vi "Mode Registration.vi"(8 "error in":errorcluster, 9 "mode":T1=-1 items=["Digital Input"=0, "Digital Output"=1, "Analog Input"=2, "PWM Input"=3, "PWM Output"=4, "Counter Rising"=5, "Counter Falling"=6, "Quadrature"=7, "Addressable LEDs"=13], 10 "device ID":i32=-1, 11 "Action":enum16{"Get", "Set", "Force", "Clear"}(ring)) -> (0 "error out":errorcluster, 2 "mode out":T1 items=["Digital Input"=0, "Digital Output"=1, "Analog Input"=2, "PWM Input"=3, "PWM Output"=4, "Counter Rising"=5, "Counter Falling"=6, "Quadrature"=7, "Addressable LEDs"=13])   [LabVIEW 2023]
uses:
  <vilib>/MRC/Types/MRC Smart IO Mode.ctl
  <vilib>/MRC/MrcLib.lvlib
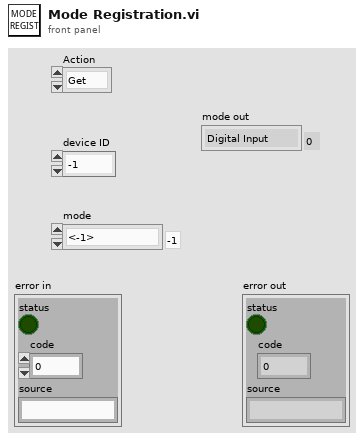
[diagram p1: front panel]
types:
  T1 = typedef "MRC Smart IO Mode.ctl" = i32
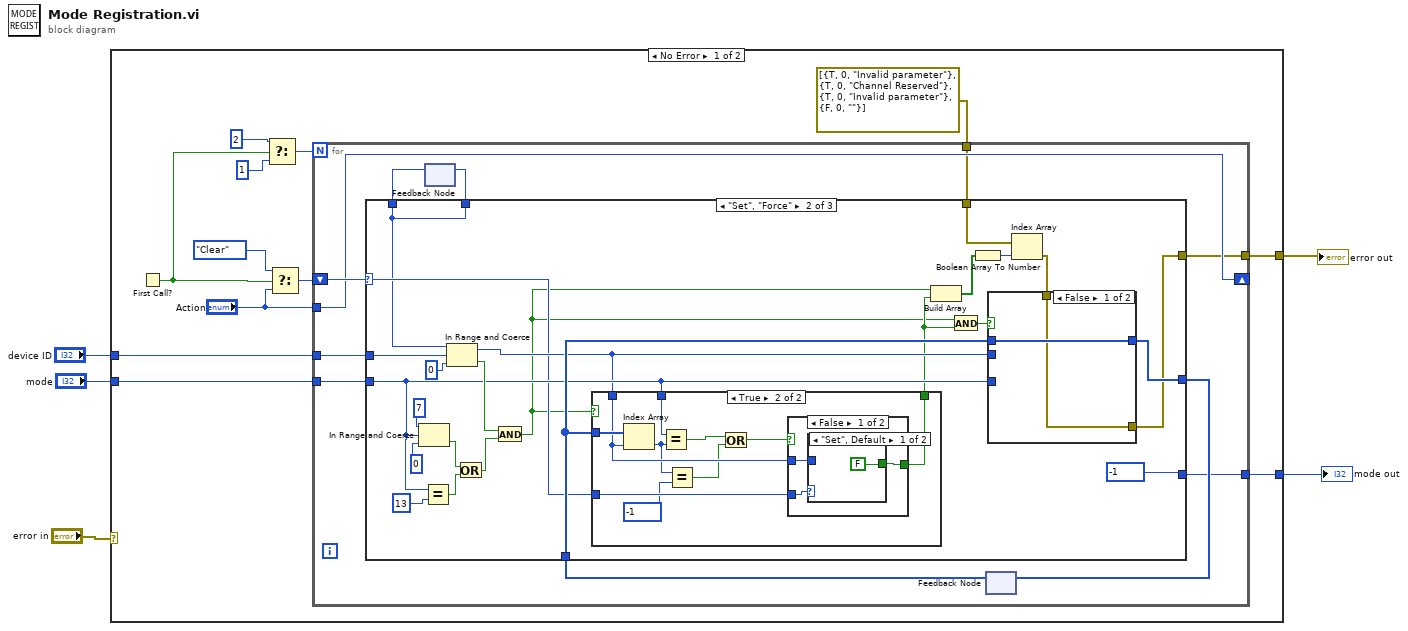
[diagram p0: block diagram]
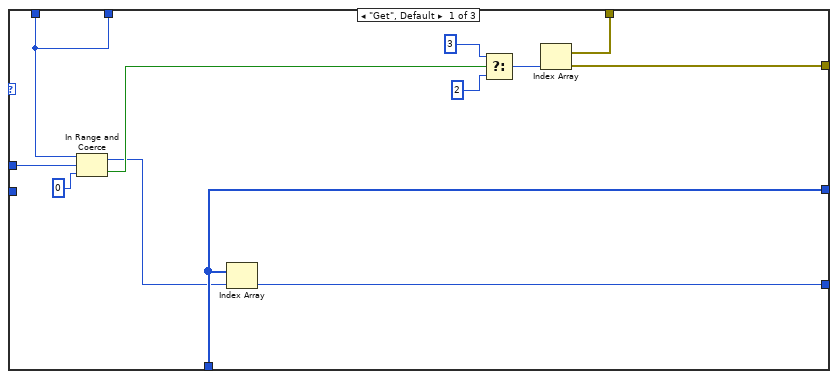
[diagram p2: hidden frame]
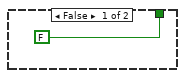
[diagram p3: hidden frame]
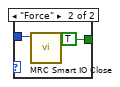
[diagram p4: hidden frame]
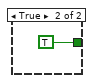
[diagram p5: hidden frame]
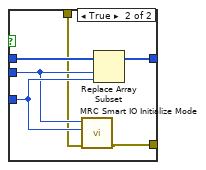
[diagram p6: hidden frame]
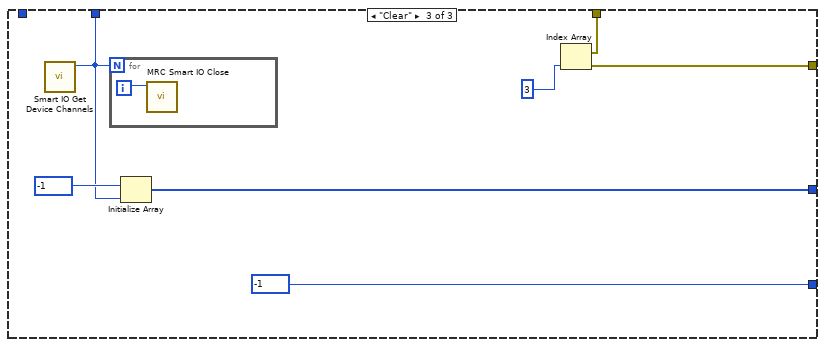
[diagram p7: hidden frame]
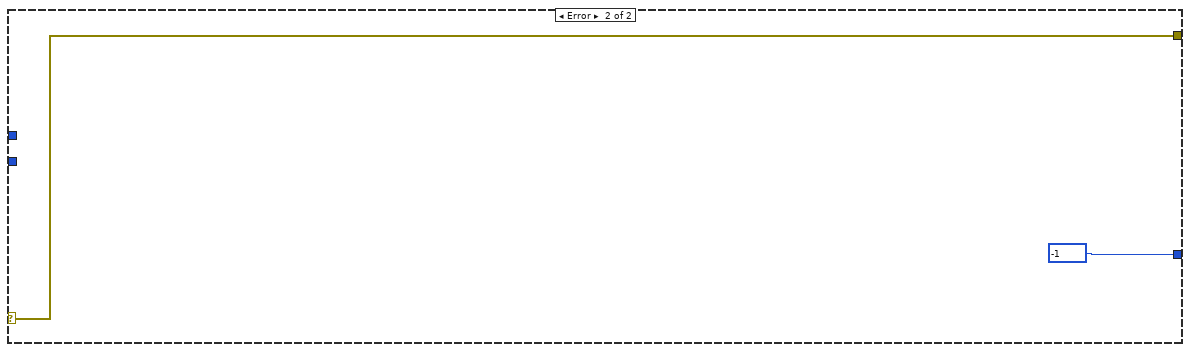
[diagram p8: hidden frame]
diagram:
  n1 = case shown="No Error" "error in" {
    selector: "error in" -> [_ w100]
    tunnel: "device ID" -> [w17 _]
    tunnel: "mode" -> [w16 _]
    tunnel: [w13 w99] -> w3
    tunnel: [w7 w100] -> w2
    frame No Error {
      n2 = First Call?() -> (First Call?: T/F=w12:bool)
      n3 = Select(t=2, s=w12, f=1) -> (s? t:f=w9:i32)
      n4 = Select(t=enum16{"Get", "Set", "Force", "Clear"}."Clear" ("y"), s=w12, f="Action") -> (s? t:f=w14:enum16{"Get", "Set", "Force", "Clear"})
      n5 = for {
        N: w9 -> [_]
        tunnel: w17 -> [w25]
        tunnel: w16 -> [w24]
        tunnel: [w21] -> w13
        shift-right: [w20] -> _
        shift-left: w14 -> [w23]
        tunnel: "Action" -> [w20]
        tunnel: [w19] -> w7
        tunnel: errorcluster[] [{"status"=TRUE, "code"=0, "source"="Invalid parameter"}, {"status"=TRUE, "code"=0, "source"="Channel Reserved"}, {"status"=TRUE, "code"=0, "source"="Invalid parameter"}, {"status"=FALSE, "code"=0, "source"=""}] -> [w18]
        n6 = feedback #1() -> (w26:i32)  [unwired: 1 in]
        n7 = feedback #2() -> (w28:T1[])  [unwired: 1 in]
        n8 = case shown="\"Set\", \"Force\"" w23 {
          selector: w23 -> [_ w51 _]
          tunnel: [w38 w57 w96] -> w22
          tunnel: w28 -> [w38 w54 _]
          tunnel: [w29 w41 w94] -> w27
          tunnel: w26 -> [w29 w41 _]
          tunnel: w25 -> [w40 w56 _]
          tunnel: w24 -> [_ w53 _]
          tunnel: [w36 w55 w95] -> w21
          tunnel: [w31 w43 w93] -> w19
          tunnel: w18 -> [w33 w45 w92]
          frame "Get", Default {
            # "Check input params"
            n9 = In Range and Coerce(upper limit=w29, x=w40, lower limit=0 ("upper limit")) -> (coerced(x)=w37:i32, In Range?=w39:bool)
            n10 = Index Array(array=w38, index=w37) -> (element=w36:T1)
            n11 = Select(t=3, s=w39, f=2) -> (s? t:f=w32:i32)
            n12 = Index Array(array=w33, index=w32) -> (element=w31:errorcluster)
          }
          frame "Set", "Force" {
            w55 = T1 -1 items=["Digital Input"=0, "Digital Output"=1, "Analog Input"=2, "PWM Input"=3, "PWM Output"=4, "Counter Rising"=5, "Counter Falling"=6, "Quadrature"=7, "Addressable LEDs"=13] ("mode")
            # "Check input params"
            n13 = In Range and Coerce(upper limit=7, x=w53, lower limit=0 ("upper limit")) -> (In Range?=w60:bool)  [unwired: 1 out]
            n14 = Equal?(x=w53, y=13 ("upper limit")) -> (x = y?=w61:bool)
            n15 = In Range and Coerce(upper limit=w41, x=w56, lower limit=0 ("upper limit")) -> (coerced(x)=w52:i32, In Range?=w59:bool)
            n16 = Or(x=w60, y=w61) -> (x .or. y?=w58:bool)
            n17 = And(x=w59, y=w58) -> (x .and. y?=w48:bool)
            n18 = case shown="True" w48 {
              tunnel: w54 -> [_ w75]
              tunnel: w53 -> [_ w74]
              tunnel: w52 -> [_ w72]
              tunnel: w51 -> [_ w71]
              tunnel: [FALSE w70] -> w49
              frame False {
              }
              frame True {
                w67 = T1 -1 items=["Digital Input"=0, "Digital Output"=1, "Analog Input"=2, "PWM Input"=3, "PWM Output"=4, "Counter Rising"=5, "Counter Falling"=6, "Quadrature"=7, "Addressable LEDs"=13] ("y")
                n19 = Index Array(array=w75, index=w72) -> (element=w68:T1)
                n20 = Equal?(x=w74, y=w68) -> (x = y?=w73:bool)
                n21 = Equal?(x=w68, y=w67) -> (x = y?=w66:bool)
                n22 = Or(x=w73, y=w66) -> (x .or. y?=w69:bool)
                n23 = case shown="False" w69 {
                  tunnel: w72 -> [w78 _]
                  tunnel: w71 -> [w77 _]
                  tunnel: [w76 TRUE] -> w70
                  frame False {
                    n24 = case shown="\"Set\", Default" w77 {
                      tunnel: w78 -> [_ w81]
                      tunnel: [FALSE TRUE] -> w76
                      frame "Set", Default {
                      }
                      frame "Force" {
                        n25 = call <vilib>:"MRC Smart IO Close.vi"("deviceIndex"=w81) -> ()  [unwired: 10 in, 1 out]
                      }
                    }
                  }
                  frame True {
                  }
                }
              }
            }
            n26 = Build Array(w48, w49) -> (w47:bool[])
            n27 = And(x=w48, y=w49) -> (x .and. y?=w50:bool)
            n28 = Boolean Array To Number(Boolean array=w47) -> (number=w46:u32)
            n29 = Index Array(array=w45, index=w46) -> (element=w44:errorcluster)
            n30 = case shown="False" w50 {
              tunnel: w54 -> [w84 w90]
              tunnel: [w84 w89] -> w57
              tunnel: w53 -> [_ w88]
              tunnel: w52 -> [_ w87]
              tunnel: w44 -> [w83 w86]
              tunnel: [w83 w85] -> w43
              frame False {
              }
              frame True {
                n31 = call <vilib>:"MRC Smart IO Initialize Mode.vi"("error in (no error)"=w86, "mode"=w88, "deviceIndex"=w87) -> ("error out"=w85:errorcluster)  [unwired: 8 in]
                n32 = Replace Array Subset(array=w90, new element=w88, index=w87) -> (w89:T1[])
              }
            }
          }
          frame "Clear" {
            w95 = T1 -1 items=["Digital Input"=0, "Digital Output"=1, "Analog Input"=2, "PWM Input"=3, "PWM Output"=4, "Counter Rising"=5, "Counter Falling"=6, "Quadrature"=7, "Addressable LEDs"=13] ("mode")
            w97 = T1 -1 items=["Digital Input"=0, "Digital Output"=1, "Analog Input"=2, "PWM Input"=3, "PWM Output"=4, "Counter Rising"=5, "Counter Falling"=6, "Quadrature"=7, "Addressable LEDs"=13] ("mode")
            n33 = call <vilib>:"Smart IO Get Device Channels.vi"() -> ("device count"=w94:i32)  [unwired: 10 in, 1 out]
            n34 = for {
              N: w94 -> [_]
              i -> [w98]
              n35 = call <vilib>:"MRC Smart IO Close.vi"("deviceIndex"=w98) -> ()  [unwired: 10 in, 1 out]
            }
            n36 = Initialize Array(w97, w94) -> (w96:T1[])
            n37 = Index Array(array=w92, index=3) -> (element=w93:errorcluster)
          }
        }
        n38 = feedback-in #1(w27) -> ()
        n39 = feedback-in #2(w22) -> ()
      }
    }
    frame Error {
      w99 = T1 -1 items=["Digital Input"=0, "Digital Output"=1, "Analog Input"=2, "PWM Input"=3, "PWM Output"=4, "Counter Rising"=5, "Counter Falling"=6, "Quadrature"=7, "Addressable LEDs"=13] ("mode")
    }
  }
  "mode out" <- w3
  "error out" <- w2
